vi "Compass read.vi"() -> ()   [LabVIEW 2013]
uses:
  <vilib>/Instr/_visa.llb/VISA Configure Serial Port (Instr).vi
panel:
  out "output cluster":cluster{dbl, dbl, dbl}(graph)
  in  "Stop Button":bool
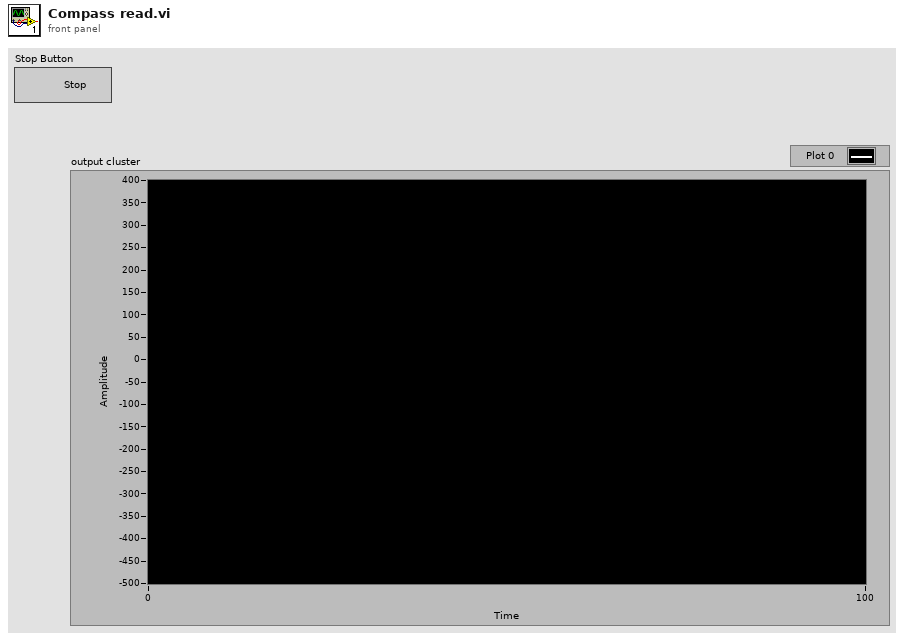
[diagram p1: front panel]
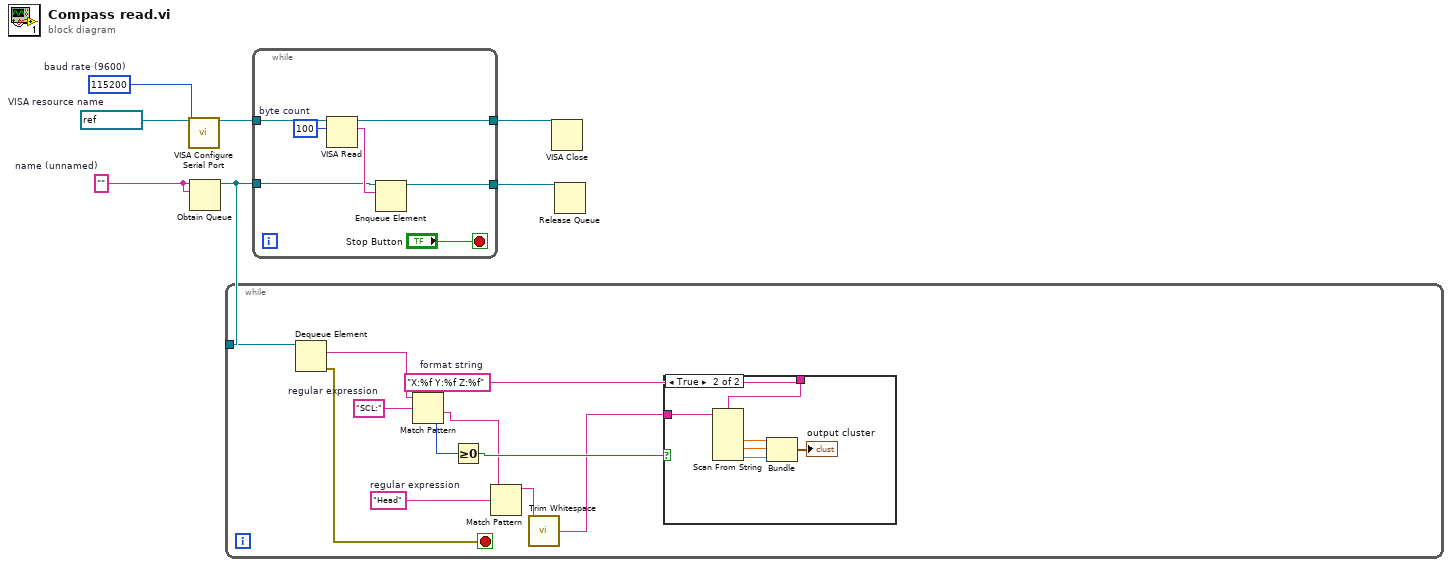
[diagram p0: block diagram]
diagram:
  w1 = ""  # name (unnamed)
  w4 = u32 115200  # baud rate (9600)
  w5 = refnum<visa-resource-name> "COM6"  # VISA resource name
  n1 = call-poly "VISA Configure Serial Port"("VISA resource name"=w5, "baud rate (9600)"=w4) -> ("VISA resource name out"=w7:refnum<visa-resource-name>)  [unwired: 12 in, 1 out]
  n2 = Obtain Queue(name (unnamed)=w1, element data type=w1) -> (queue out=w2:refnum<queue>)  [unwired: 3 in, 2 out]
  n3 = while {
    tunnel: w2 -> [w18]
    stop <- w17 stop-if-true
    w10 = "Head"  # regular expression
    w14 = "X:%f Y:%f Z:%f"  # format string
    w15 = "SCL:"  # regular expression
    n4 = Dequeue Element(queue=w18) -> (element=w16:string, error out=w17:errorcluster)  [unwired: 2 in, 2 out]
    n5 = Match Pattern(string=w16, regular expression=w15) -> (after substring=w11:string, offset past match=w13:i32)  [unwired: 1 in, 2 out]
    n6 = Greater Or Equal To 0?(x=w13) -> (x >= 0?=w12:bool)
    n7 = Match Pattern(string=w11, regular expression=w10) -> (before substring=w9:string)  [unwired: 1 in, 3 out]
    n8 = call <vilib>:"Trim Whitespace.vi"("string"=w9) -> ("trimmed string"=w8:string)  [unwired: 1 in]
    n9 = case shown="True" w12 {
      tunnel: w8 -> [_ w24]
      tunnel: w14 -> [_ w23]
      frame False {
      }
      frame True {
        n10 = Scan From String(format string=w23, input string=w24) -> (output 1=w22:dbl, output 2=w21:dbl, output 3=w20:dbl)  [unwired: 5 in, 3 out]
        n11 = Bundle(w22, w21, w20) -> (→"output cluster":cluster{dbl, dbl, dbl})  [unwired: 1 in]
      }
    }
  }
  n12 = while {
    tunnel: w7 -> [w31]
    tunnel: [w30] -> w6
    tunnel: w2 -> [w26]
    tunnel: [w25] -> w3
    stop <- "Stop Button" stop-if-true
    w28 = u32 100  # byte count
    n13 = VISA Read(VISA resource name=w31, byte count=w28) -> (VISA resource name out=w30:refnum<visa-resource-name>, read buffer=w27:string)  [unwired: 1 in, 2 out]
    n14 = Enqueue Element(queue=w26, element=w27) -> (queue out=w25:refnum<queue>)  [unwired: 2 in, 2 out]
  }
  n15 = VISA Close(VISA resource name=w6) -> ()  [unwired: 1 in, 1 out]
  n16 = Release Queue(queue=w3) -> ()  [unwired: 2 in, 3 out]
